vi "Init Read Test.vi"(8 "error in (no error)":errorcluster, 10 "signal list":refnum<k21>[](array[refnum]), 11 "interface":refnum<k21>) -> (0 "error out":errorcluster, 3 "session out":refnum<k21>)   [LabVIEW 2023]
uses:
  <resource>/objmgr/xnet.rc
  <vilib>/xnet/xnet.llb/XNET Create Session (Signal Input Single-point).vi
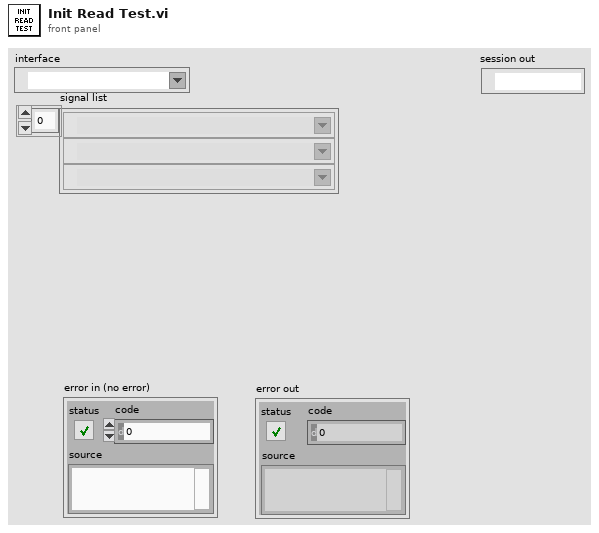
[diagram p1: front panel]
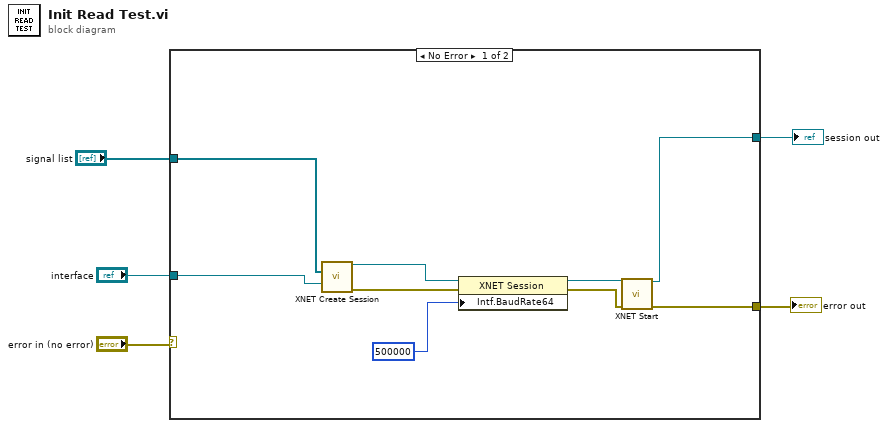
[diagram p0: block diagram]
diagram:
  n1 = case shown="No Error" "error in (no error)" {
    selector: "error in (no error)" -> [_ w15]
    tunnel: "signal list" -> [w11 _]
    tunnel: "interface" -> [w10 _]
    tunnel: [w8 w15] -> w2
    tunnel: [w6 _] -> w1
    frame No Error {
      n2 = call-poly <vilib>:"XNET Create Session.vi"("signal list"=w11, "interface"=w10) -> ("session out"=w13:refnum<k21>, "error out"=w14:errorcluster)  [unwired: 12 in]
      n3 = property class="XNET Session"(reference=w13, error in=w14, "Intf.BaudRate64"=u64 500000 ("Interface:64bit Baud Rate")) -> (reference out=w9:refnum<k21>, error out=w7:errorcluster)
      n4 = call <vilib>:"XNET Start.vi"("session in"=w9, "error in (no error)"=w7) -> ("session out"=w6:refnum<k21>, "error out"=w8:errorcluster)  [unwired: 12 in]
    }
    frame Error {
    }
  }
  "error out" <- w2
  "session out" <- w1
